vi "ASD BL estimation VI.vi"(8 "BL Selection":T4(ring), 9 "STD Cut":i32=15, 11 "Region raw data":dbl[](array[numeric])) -> (0 "Selected Region Baseline":dbl, 1 "Region BL selct":string, 2 "HPeak Cluster":T1, 3 "BL cluster":T3)   [LabVIEW 2018]
uses:
  <vilib>/Analysis/baseanly.llb/Mean (DBL).vi
  <vilib>/Analysis/baseanly.llb/Unimode.vi
  <vilib>/Analysis/NI_AALBase.lvlib
  <vilib>/Analysis/NI_AAL_SigProc.lvlib
  <vilib>/gmath/NI_Gmath.lvlib
panel:
  out "# found 2":i32 caption="検出数"
  out "Locations":dbl[](array[numeric]) caption="位置"
  out "# found":i32 caption="検出数"
  out "Histogram Graph 2":T2(graph)
  out "All Value Mode":dbl caption="モード"
  out "Div Value Mode":dbl caption="Div STD Mode (pA)"
  out "Potential Baseline":dbl
  out "# Peak Locations":dbl[](array[numeric]) caption="H Peak Location"
  out "Histogram: h(x)":i32[](array[numeric]) caption="Histogram:h(x)"
  out "H Peak#":i32 caption="H Peak #"
  out "Histogram Graph":T2(graph)
  out "Div mean value":dbl caption="Div STD  Mean (pA)"
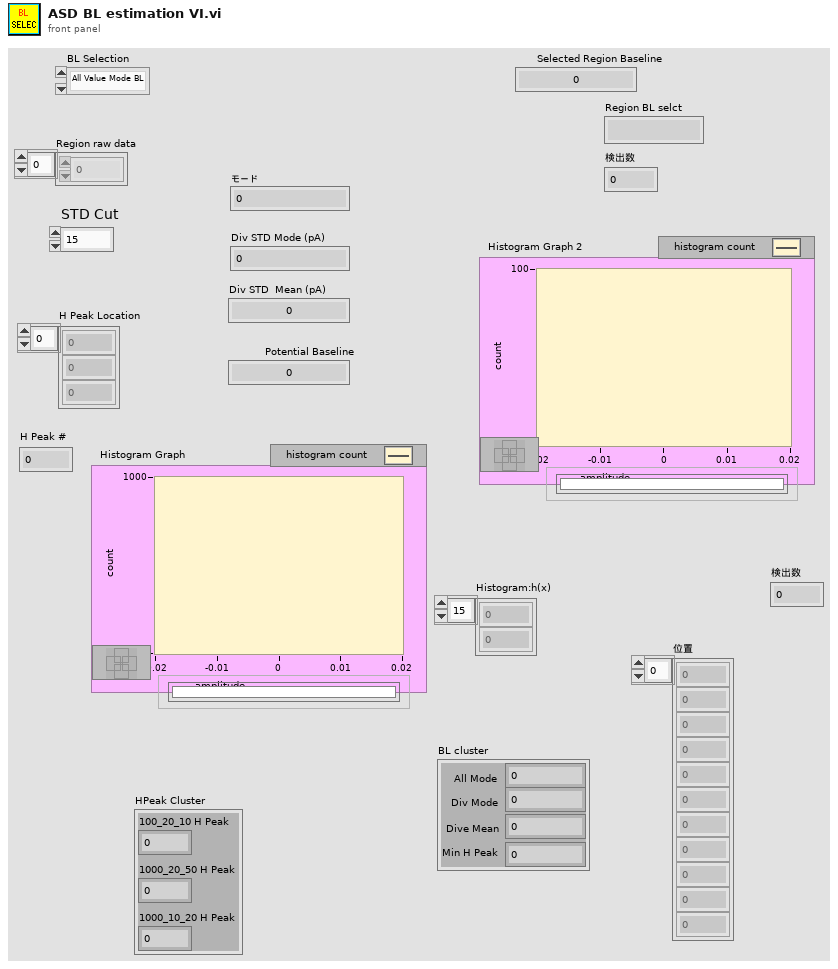
[diagram p1: front panel]
types:
  T1 = cluster{"100_20_10 H Peak":i32, "1000_20_50 H Peak":i32, "1000_10_20 H Peak":i32}
  T2 = cluster{"X Values":dbl[], "Histogram: h(x)":i32[]}
  T3 = cluster{"All Mode":dbl, "Div Mode":dbl, "Dive Mean":dbl, "Min H Peak":dbl}
  T4 = enum16{"All Value Mode BL", "Div Value Mode BL", "Div Mean Mean BL", "Min Peak Value BL"}
  T5 = cluster{"# found":i32, "# found":i32, "# found":i32}
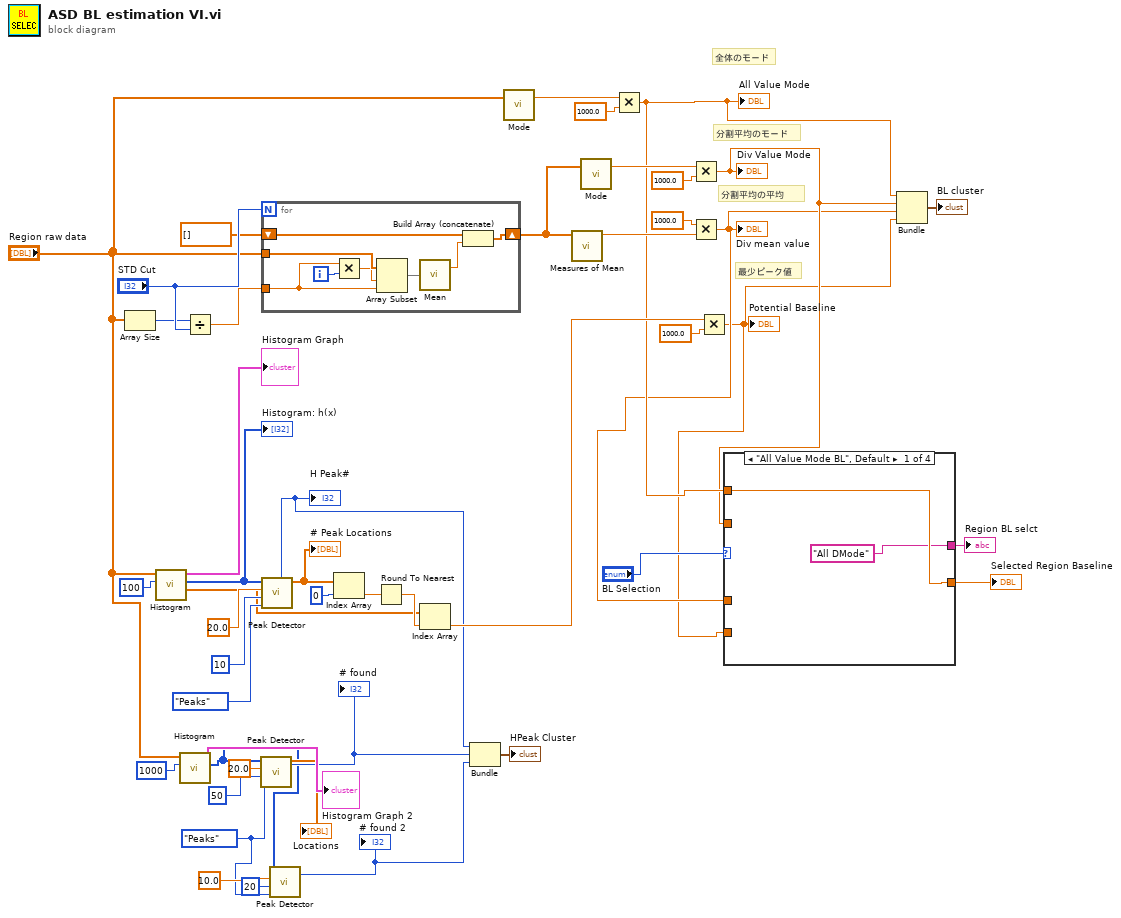
[diagram p0: block diagram]
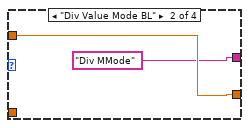
[diagram p2: hidden frame]
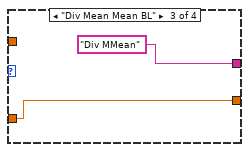
[diagram p3: hidden frame]
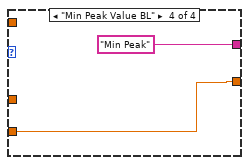
[diagram p4: hidden frame]
diagram:
  w4 = enum32{"Peaks", "Valleys"}."Peaks" ("peaks/valleys")
  # "全体のモード"
  # "分割平均のモード"
  # "分割平均の平均"
  # "最少ピーク値"
  n1 = Array Size(array="Region raw data") -> (size(s)=w41:i32)
  n2 = call <vilib>:"Histogram.vi"("intervals"=100, "X"="Region raw data") -> ("X Values"=w30:dbl[], "Histogram: h(x)"=w37:i32[], "Histogram Graph"=→"Histogram Graph":T2)  [unwired: 6 in, 1 out]
  "Histogram: h(x)" <- w37
  n3 = call <vilib>:"Histogram.vi"("intervals"=1000, "X"="Region raw data") -> ("Histogram: h(x)"=w7:i32[], "Histogram Graph"=→"Histogram Graph 2":T2)  [unwired: 6 in, 2 out]
  n4 = Divide(x=w41, y="STD Cut") -> (x/y=w46:dbl)
  n5 = call <vilib>:"Peak Detector.vi"("peaks/valleys"=w4, "width"=50, "threshold"=20.0, "X"=w7) -> ("Locations"=→"Locations":dbl[], "# found"=w8:i32)  [unwired: 3 in, 3 out]
  "# found" <- w8
  n6 = for {
    N: "STD Cut" -> [_]
    tunnel: "Region raw data" -> [w54]
    tunnel: w46 -> [w53]
    shift-right: [w48] -> w25
    shift-left: dbl[] [] -> [w47]
    i -> [w52]
    n7 = Multiply(x=w53, y=w52) -> (x*y=w51:dbl)
    n8 = Array Subset(array=w54, index=w51, length=w53) -> (w50:dbl[])
    n9 = call-poly <vilib>:"Mean.vi"("X"=w50) -> ("mean"=w49:dbl)  [unwired: 1 out]
    n10 = Build Array (concatenate)(w47, w49) -> (w48:dbl[])
  }
  n11 = call <vilib>:"Peak Detector.vi"("peaks/valleys"=enum32{"Peaks", "Valleys"}."Peaks", "width"=10, "threshold"=20.0, "X"=w37) -> ("Locations"=w34:dbl[], "# found"=w9:i32)  [unwired: 3 in, 3 out]
  "H Peak#" <- w9
  "# Peak Locations" <- w34
  n12 = call <vilib>:"Peak Detector.vi"("peaks/valleys"=w4, "width"=20, "threshold"=10.0, "X"=w7) -> ("# found"=w3:i32)  [unwired: 3 in, 4 out]
  "# found 2" <- w3
  n13 = Index Array(array=w34, index=0 ("指標")) -> (element=w32:dbl)
  n14 = Round To Nearest(number=w32) -> (nearest integer value=w31:dbl)
  n15 = Index Array(array=w30, index=w31) -> (element=w29:dbl)
  n16 = Bundle("# found"=w9, "# found"=w8, "# found"=w3) -> (→"HPeak Cluster":T5)  [unwired: 1 in]
  n17 = call-poly <vilib>:"Mode.vi"("X"="Region raw data") -> ("mode"=w24:dbl)  [unwired: 1 in, 1 out]
  n18 = call <vilib>:"Measures of Mean.vi"("x array"=w25) -> ("mean value"=w43:dbl)  [unwired: 9 in, 1 out]
  n19 = call-poly <vilib>:"Mode.vi"("X"=w25) -> ("mode"=w27:dbl)  [unwired: 1 in, 1 out]
  n20 = Multiply(x=w24, y=1000.0 ("x")) -> (x*y=w20:dbl)
  "All Value Mode" <- w20
  n21 = Multiply(x=w27, y=1000.0 ("x")) -> (x*y=w19:dbl)
  "Div Value Mode" <- w19
  n22 = Multiply(x=1000.0, y=w43) -> (x*y=w18:dbl)
  "Div mean value" <- w18
  n23 = Multiply(x=w29, y=1000.0) -> (x*y=w17:dbl)
  "Potential Baseline" <- w17
  n24 = case shown="\"All Value Mode BL\", Default" "BL Selection" {
    tunnel: [w56 w58 w60 w62] -> w21
    tunnel: w19 -> [_ w58 _ _]
    tunnel: w20 -> [w56 _ _ _]
    tunnel: w18 -> [_ _ w60 _]
    tunnel: w17 -> [_ _ _ w62]
    tunnel: ["All DMode" "Div MMode" "Div MMean" "Min Peak"] -> w15
    frame "All Value Mode BL", Default {
    }
    frame "Div Value Mode BL" {
    }
    frame "Div Mean Mean BL" {
    }
    frame "Min Peak Value BL" {
    }
  }
  "Selected Region Baseline" <- w21
  "Region BL selct" <- w15
  n25 = Bundle(w20, w19, w18, w17) -> (→"BL cluster":cluster{dbl, dbl, dbl, dbl})  [unwired: 1 in]
